vi "Script RPC Client VI.vi"(6 "rpc method parameters":T1, 7 "owning library":refnum<vi>, 8 "error in (no error)":errorcluster, 9 "rpc service name":string, 10 "owning folder":refnum<vi>, 11 "template project item":refnum<vi>) -> (0 "error out":errorcluster)   [LabVIEW 2019, in "gRPC Template Creation Utility.lvlib"]
uses:
  gRPC Template Creation Utility.lvlib
  TypeDefs/RPC Method Parameters.ctl
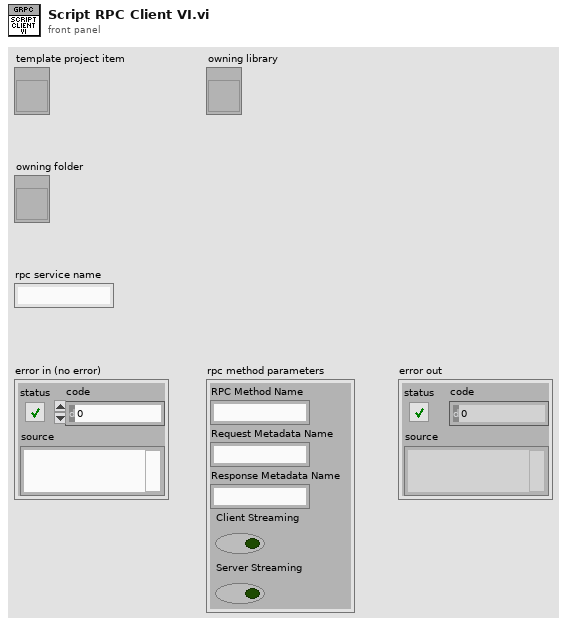
[diagram p1: front panel]
types:
  T1 = typedef "gRPC Template Creation Utility.lvlib/RPC Method Parameters.ctl" = cluster{"RPC Method Name":string, "Request Metadata Name":string, "Response Metadata Name":string, "Client Streaming":bool, "Server Streaming":bool}
  T2 = enum32{"invalid VI type", "Standard VI", "Control VI", "Global VI", "Polymorphic VI", "Configuration VI", "SubSystem", "Facade VI", "Method VI"}
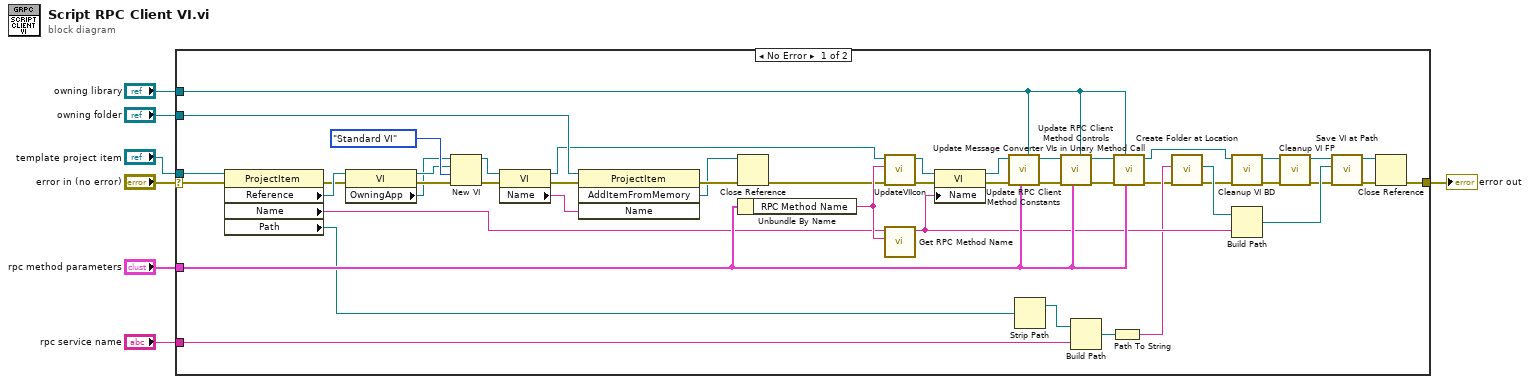
[diagram p0: block diagram]
diagram:
  n1 = case shown="No Error" "error in (no error)" {
    selector: "error in (no error)" -> [w27 w55]
    tunnel: "rpc method parameters" -> [w54 _]
    tunnel: "owning library" -> [w53 _]
    tunnel: [w26 w55] -> w5
    tunnel: "rpc service name" -> [w41 _]
    tunnel: "owning folder" -> [w39 _]
    tunnel: "template project item" -> [w30 _]
    frame No Error {
      n2 = property class="ProjectItem"(reference=w30, error in=w27) -> (error out=w11:errorcluster, "Reference"=w12:refnum<vi>, "Name"=w29:string, "Path"=w28:path)  [unwired: 1 out]
      n3 = property class="VI"(reference=w12, error in=w11) -> (reference out=w9:refnum<vi>, error out=w10:errorcluster, "OwningApp"=w8:refnum<vi>)
      n4 = New VI(8:w10, 9:T2."Standard VI" ("vi type (standard vi)"), 10:w9, 11:w8) -> (0:w24:errorcluster, 3:w25:refnum<vi>)  [unwired: 3 out]
      n5 = property class="VI"(reference=w25, error in=w24) -> (reference out=w23:refnum<vi>, error out=w33:errorcluster, "Name"=w31:string)
      n6 = invoke class="ProjectItem" method="AddItemFromMemory"(reference=w39, error in=w33, "Name"=w31) -> (error out=w38:errorcluster, "AddItemFromMemory"=w37:refnum<vi>)  [unwired: 1 in, 2 out]
      n7 = Close Reference(reference=w37, error in (no error)=w38) -> (error out=w20:errorcluster)
      n8 = Unbundle By Name(w54) -> ("RPC Method Name"=w50:string)
      n9 = call "UpdateVIIcon.vi"("error in (no error)"=w20, "Method Name"=w50, "VI in"=w23) -> ("error out"=w21:errorcluster, "VI out"=w22:refnum<vi>)  [unwired: 7 in]
      n10 = call "Get RPC Method Name.vi"("RPC Method Name"=w50, "Template VI Name"=w29) -> ("RPC VI Name"=w49:string)  [unwired: 8 in, 1 out]
      n11 = property class="VI"(reference=w22, error in=w21, "Name"=w49) -> (reference out=w47:refnum<vi>, error out=w45:errorcluster)
      n12 = call "Update RPC Client Method Constants.vi"("Library"=w53, "RPC Method Parameters"=w54, "error in (no error)"=w45, "VI in"=w47) -> ("error out"=w46:errorcluster, "VI out"=w48:refnum<vi>)  [unwired: 6 in]
      n13 = Strip Path(path=w28) -> (stripped path=w40:path)  [unwired: 1 out]
      n14 = call "Update RPC Client Method Controls.vi"("Library"=w53, "RPC Method Parameters"=w54, "error in (no error)"=w46, "VI in"=w48) -> ("error out"=w52:errorcluster, "VI out"=w51:refnum<vi>)  [unwired: 6 in]
      n15 = Build Path(base path=w40, name or relative path=w41) -> (appended path=w42:path)
      n16 = Path To String(path=w42) -> (string=w43:string)
      n17 = call "Update Message Converter VIs in Unary Method Call.vi"("RPC Method Parameters"=w54, "Library"=w53, "error in (no error)"=w52, "VI in"=w51) -> ("error out"=w19:errorcluster, "VI out"=w16:refnum<vi>)  [unwired: 6 in]
      n18 = call "Create Folder at Location.vi"("Error In"=w19, "Path"=w43) -> ("Error Out"=w14:errorcluster, "Full path out"=w44:path)  [unwired: 7 in, 1 out]
      n19 = call "Cleanup VI BD.vi"("error in (no error)"=w14, "VI in"=w16) -> ("error out"=w18:errorcluster, "VI out"=w17:refnum<vi>)  [unwired: 8 in]
      n20 = Build Path(base path=w44, name or relative path=w49) -> (appended path=w34:path)
      n21 = call "Cleanup VI FP.vi"("error in"=w18, "vi in"=w17) -> ("error out"=w13:errorcluster, "vi out"=w15:refnum<vi>)  [unwired: 8 in]
      n22 = call "Save VI at Path.vi"("error in (no error)"=w13, "Path"=w34, "VI in"=w15) -> ("error out"=w35:errorcluster, "VI out"=w36:refnum<vi>)  [unwired: 6 in, 1 out]
      n23 = Close Reference(reference=w36, error in (no error)=w35) -> (error out=w26:errorcluster)
    }
    frame Error {
    }
  }
  "error out" <- w5
